vi "Module Init.vi"(8 "error in (no error)":errorcluster, 11 "DAQmxDO in":refnum<class "DAQmxDO.lvclass">) -> (0 "error out":errorcluster, 3 "DAQmxDO out":refnum<class "DAQmxDO.lvclass">)   [LabVIEW 2020, in "VolatusDAQ.lvlib" / "DAQmxDO.lvclass"]
uses:
  DAQmxDO.lvclass
  C:/dev/lv20CE/relink/lv-volatus/Volatus/Module/Module.lvclass
  Volatus/Message Registration.ctl
  VolatusData/DataProc Options.ctl
  DAQmxDO.lvclass/DAQmxDO.ctl
  Volatus/Module/Module.lvclass/Module.ctl
  Volatus/MessageQ/MessageQ.lvclass/MessageQ.ctl
  Volatus/Module/Self Q.vi
  Volatus/MessageQ/Send.vi
  Volatus/Module/Module.lvclass
  VolatusData/Data Processor Module/Data Processor Module.lvclass
  VolatusDAQ.lvlib
  Volatus/Volatus.lvlib
  VolatusData/VolatusData.lvlib
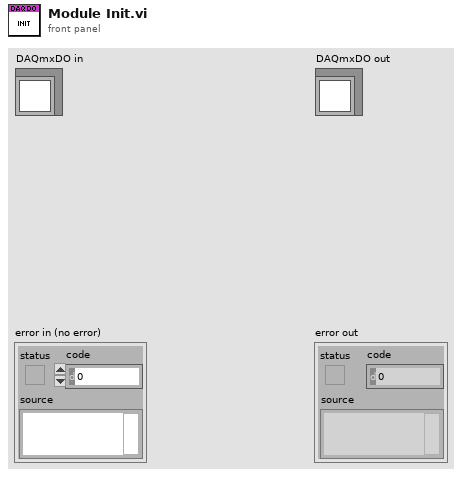
[diagram p1: front panel]
types:
  T1 = typedef "VolatusData.lvlib/DataProc Options.ctl" = cluster{"Ignore Scaling":bool}
  T2 = typedef "Volatus.lvlib/Message Registration.ctl" = cluster{"Message Type":string, "Message ID":string}
  T3 = typedef "VolatusDAQConfig.lvlib/Sampling Config.ctl" = cluster{"Rate":dbl, "Chunk Size":i32}
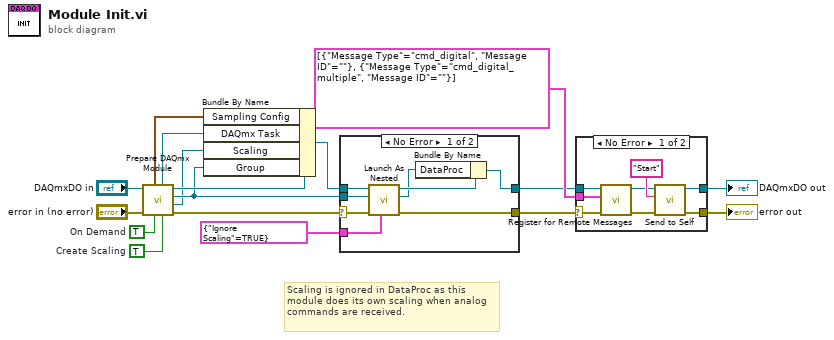
[diagram p0: block diagram]
diagram:
  w6 = TRUE  # On Demand
  w7 = TRUE  # Create Scaling
  # "Scaling is ignored in DataProc as this module does its own scaling when analog commands are received."
  n1 = call "Prepare DAQmx Module.vi"("Create Scaling (F)"=w7, "On Demand (F)"=w6, "error in (no error)"="error in (no error)", "Module in"="DAQmxDO in") -> ("error out"=w14:errorcluster, "Scaling"=w11:refnum<class "Scaling.lvclass">, "Group"=w12:refnum<class "Group.lvclass">, "Module out"=w17:refnum<class "DAQmxDO.lvclass">, "DAQmx Task"=w16:refnum<k21>, "Sampling Config"=w15:T3)  [unwired: 2 in]
  n2 = Bundle By Name(cluster=w17, "Sampling Config"=w15, "DAQmx Task"=w16, "Scaling"=w11, "Group"=w12) -> (w13:refnum<class "DAQmxDO.lvclass">)
  n3 = case shown="No Error" w14 {
    selector: w14 -> [w25 w26]
    tunnel: w13 -> [w24 w27]
    tunnel: w12 -> [w23 _]
    tunnel: [w22 w26] -> w8
    tunnel: [w19 w27] -> w9
    tunnel: T1 {"Ignore Scaling"=TRUE} ("DataProc Options") -> [w18 _]
    frame No Error {
      n4 = call "Launch As Nested.vi"("DataProc Options"=w18, "error in (no error)"=w25, "Group"=w23, "Parent in"=w24) -> ("error out"=w22:errorcluster, "MessageQ"=w20:refnum<class "MessageQ.lvclass">, "Parent out"=w21:refnum<class "DAQmxDO.lvclass">)  [unwired: 5 in]
      n5 = Bundle By Name(cluster=w21, "DataProc"=w20) -> (w19:refnum<class "DAQmxDO.lvclass">)
    }
    frame Error {
    }
  }
  n6 = case shown="No Error" w8 {
    selector: w8 -> [w30 w37]
    tunnel: [w35 w37] -> w2
    tunnel: w9 -> [w31 w36]
    tunnel: [w34 w36] -> w3
    tunnel: T2[] [{"Message Type"="cmd_digital", "Message ID"=""}, {"Message Type"="cmd_digital_multiple", "Message ID"=""}] ("Messages") -> [w32 _]
    frame No Error {
      n7 = call "Register for Remote Messages.vi"("error in (no error)"=w30, "Messages"=w32, "Module in"=w31) -> ("error out"=w28:errorcluster, "Module out"=w29:refnum<class "DAQmxDO.lvclass">)  [unwired: 7 in]
      n8 = call "Send to Self.vi"("error in (no error)"=w28, "Message ID"="Start", "Module in"=w29) -> ("error out"=w35:errorcluster, "Module out"=w34:refnum<class "DAQmxDO.lvclass">)  [unwired: 7 in]
    }
    frame Error {
    }
  }
  "error out" <- w2
  "DAQmxDO out" <- w3
